vi "Load Sequence.vi"(8 "error in":errorcluster, 10 "path":path, 11 "Sequence Executor in":refnum<class "Sequence Executor.lvclass">) -> (0 "error out":errorcluster, 3 "Sequence Executor out":refnum<class "Sequence Executor.lvclass">)   [LabVIEW 2026, in "Sequence Executor.lvclass"]
doc: "Loads a sequence JSON and launches its rig plug-in. Refuses while Running. Reads and parses the sequence and rig config and validates them; any error or invalid sequence sets Status LOAD ERROR and returns NO error (AF would stop the actor). Otherwise stops the previous rig, loads the plug-in class, casts it to Rig, sets its config, launches it nested (auto-stop), and stores Sequence, Rig Config, Rig Enqueuer, Loaded, Results (all NOT RUN) and Status through the class accessors. A launch error also sets Status LOAD ERROR and Loaded F."
uses:
  Sequence Executor.lvclass
  Rig/Rig.lvclass
  Sequence Executor.lvclass/Sequence Executor.ctl
  <vilib>/ActorFramework/Message Enqueuer/Message Enqueuer.lvclass/Message Enqueuer.ctl
  <vilib>/ActorFramework/Message Enqueuer/Enqueue.vi
  <vilib>/ActorFramework/Stop Msg/Stop Msg.lvclass
  <vilib>/ActorFramework/Message Priority Queue/Priority Enqueue.vi
  <vilib>/ActorFramework/Message Enqueuer/Message Enqueuer.lvclass
  <vilib>/ActorFramework/Actor/Actor.lvclass
panel:
  in  "Rig type":refnum<class "Rig.lvclass">
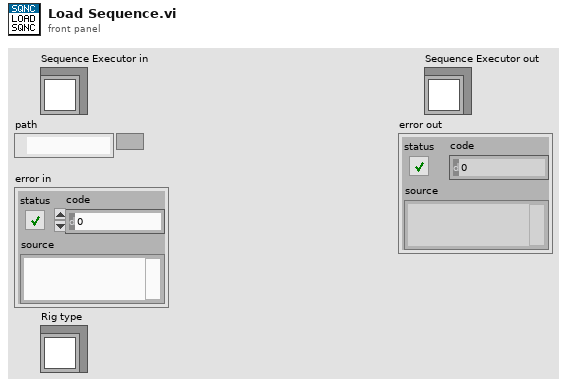
[diagram p1: front panel]
types:
  T1 = cluster{"step_no":i32, "step_name":string, "result":string, "reason":string, "measured":dbl, "target":dbl, "duration_ms":dbl}
  T2 = typedef "Sequence File.ctl" = cluster{"sequence_id":string, "description":string, "rig_config":string, "steps":T3[]}
  T3 = typedef "Step Config.ctl" = cluster{"step_no":i32, "step_name":string, "command_type":string, "setpoints":T4[], "conditions":T5[], "dwell_time_ms":i32, "timeout_ms":i32, "expected_result":string}
  T4 = typedef "Channel Value.ctl" = cluster{"channel":string, "value":dbl}
  T5 = typedef "Condition.ctl" = cluster{"channel":string, "target":dbl, "tolerance":dbl}
  T6 = typedef "Rig Config.ctl" = cluster{"rig_id":string, "description":string, "plugin_class":string, "channels":T7[]}
  T7 = typedef "Channel Definition.ctl" = cluster{"name":string, "unit":string, "min":dbl, "max":dbl}
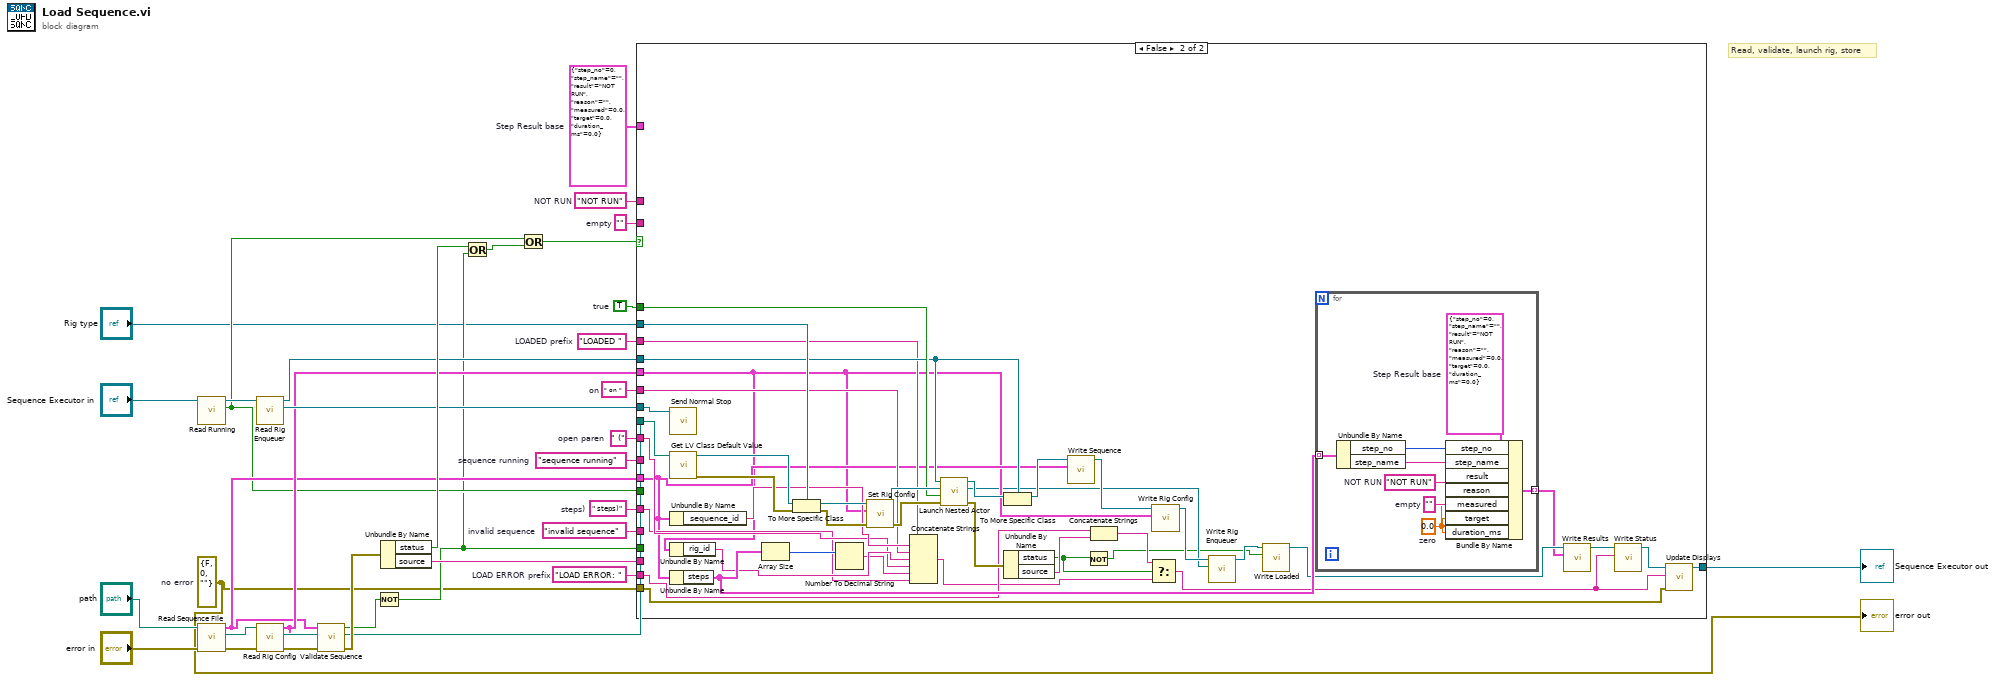
[diagram p0: block diagram]
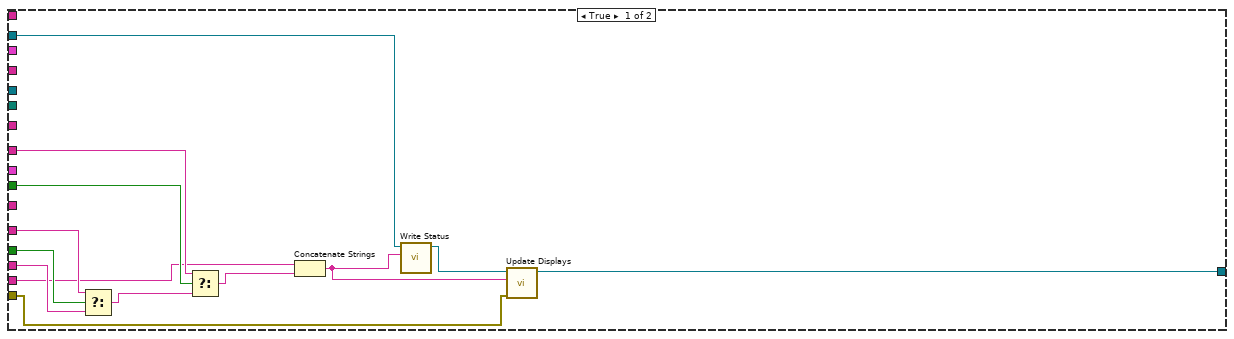
[diagram p2: hidden frame]
diagram:
  w11 = T1 {"step_no"=0, "step_name"="", "result"="NOT RUN", "reason"="", "measured"=0.0, "target"=0.0, "duration_ms"=0.0}  # Step Result base
  w12 = TRUE  # true
  w5 = " steps)"  # steps)
  w6 = " ("  # open paren
  w7 = " on "  # on
  w8 = "LOADED "  # LOADED prefix
  w9 = ""  # empty
  w10 = "NOT RUN"  # NOT RUN
  w15 = "invalid sequence"  # invalid sequence
  w14 = "sequence running"  # sequence running
  w13 = "LOAD ERROR: "  # LOAD ERROR prefix
  w3 = errorcluster {"status"=FALSE, "code"=0, "source"=""}  # no error
  # "Read, validate, launch rig, store"
  n1 = call "Read Running.vi"("Sequence Executor in"="Sequence Executor in") -> ("Running"=w17:bool, "Sequence Executor out"=w28:refnum<class "Sequence Executor.lvclass">)  [unwired: 8 in, 1 out]
  n2 = call "Read Sequence File.vi"("error in"="error in", "path"="path") -> ("error out"=w31:errorcluster, "rig config path"=w32:path, "Sequence File"=w19:T2)  [unwired: 7 in]
  n3 = call "Read Rig Enqueuer.vi"("Sequence Executor in"=w28) -> ("Actor Framework:Message Enqueuer"=w22:refnum<class "Message Enqueuer.lvclass">, "Sequence Executor out"=w23:refnum<class "Sequence Executor.lvclass">)  [unwired: 8 in, 1 out]
  n4 = call "Read Rig Config.vi"("error in"=w31, "path"=w32) -> ("error out"=w30:errorcluster, "plugin class path"=w21:path, "Rig Config"=w20:T6)  [unwired: 7 in]
  n5 = call "Validate Sequence.vi"("error in"=w30, "Rig Config"=w20, "Sequence File"=w19) -> ("error out"=w27:errorcluster, "valid"=w26:bool)  [unwired: 6 in, 1 out]
  n6 = Not(x=w26) -> (.not. x?=w16:bool)
  n7 = Unbundle By Name(w27) -> ("status"=w25:bool, "source"=w18:string)
  n8 = Or(x=w25, y=w16) -> (x .or. y?=w24:bool)
  n9 = Or(x=w17, y=w24) -> (x .or. y?=w1:bool)
  n10 = case shown="False" w1 {
    tunnel: w23 -> [w39 w78]
    tunnel: w22 -> [_ w89]
    tunnel: w21 -> [_ w88]
    tunnel: w20 -> [_ w59]
    tunnel: w19 -> [_ w61]
    tunnel: w18 -> [w45 _]
    tunnel: w17 -> [w44 _]
    tunnel: w16 -> [w47 _]
    tunnel: w15 -> [w46 _]
    tunnel: w14 -> [w43 _]
    tunnel: w13 -> [w41 w67]
    tunnel: w12 -> [_ w81]
    tunnel: w11 -> [_ _]
    tunnel: w10 -> [_ _]
    tunnel: w9 -> [_ _]
    tunnel: w8 -> [_ w75]
    tunnel: w7 -> [_ w73]
    tunnel: w6 -> [_ w71]
    tunnel: w5 -> [_ w69]
    tunnel: "Rig type" -> [_ w86]
    tunnel: w3 -> [w36 w49]
    tunnel: [w35 w48] -> w2
    frame True {
      n11 = Select(t=w46, s=w47, f=w45) -> (s? t:f=w42:string)
      n12 = Select(t=w43, s=w44, f=w42) -> (s? t:f=w40:string)
      n13 = Concatenate Strings(w41, w40) -> (w37:string)
      n14 = call "Write Status.vi"("Status"=w37, "Sequence Executor in"=w39) -> ("Sequence Executor out"=w38:refnum<class "Sequence Executor.lvclass">)  [unwired: 8 in, 1 out]
      n15 = call "Update Displays.vi"("error in"=w36, "Status"=w37, "Sequence Executor in"=w38) -> ("Sequence Executor out"=w35:refnum<class "Sequence Executor.lvclass">)  [unwired: 7 in, 1 out]
    }
    frame False {
      n16 = call <vilib>:"Send Normal Stop.vi"("Message Enqueuer"=w89) -> ()  [unwired: 10 in, 1 out]
      n17 = call <vilib>:"Get LV Class Default Value.vi"("class path"=w88) -> ("error out"=w85:errorcluster, "object"=w87:refnum<class>)  [unwired: 9 in]
      n18 = Unbundle By Name(w61) -> ("sequence_id"=w74:string)
      n19 = Unbundle By Name(w59) -> ("rig_id"=w72:string)
      n20 = Unbundle By Name(w61) -> ("steps"=w77:T3[])
      n21 = Array Size(array=w77) -> (size(s)=w76:i32)
      n22 = To More Specific Class(target class=w86, reference=w87, error in=w85) -> (specific class reference=w84:refnum<class "Rig.lvclass">, error out=w83:errorcluster)
      n23 = Number To Decimal String(number=w76) -> (decimal integer string=w70:string)  [unwired: 1 in]
      n24 = call "Set Rig Config.vi"("error in"=w83, "Rig Config"=w59, "Rig in"=w84) -> ("error out"=w80:errorcluster, "Rig out"=w82:refnum<class "Rig.lvclass">)  [unwired: 7 in]
      n25 = Concatenate Strings(w75, w74, w73, w72, w71, w70, w69) -> (w64:string)
      n26 = call <vilib>:"Launch Nested Actor.vi"("error in (no error)"=w80, "Auto-stop? (T)"=w81, "Nested Actor"=w82, "Caller Actor in"=w78) -> ("error out"=w68:errorcluster, "Nested Actor's Enqueuer"=w57:refnum<class "Message Enqueuer.lvclass">, "Caller Actor out"=w79:refnum<class "Sequence Executor.lvclass">)  [unwired: 5 in]
      n27 = To More Specific Class(target class=w78, reference=w79) -> (specific class reference=w62:refnum<class "Sequence Executor.lvclass">)  [unwired: 1 in, 1 out]
      n28 = Unbundle By Name(w68) -> ("status"=w63:bool, "source"=w66:string)
      n29 = call "Write Sequence.vi"("Sequence File"=w61, "Sequence Executor in"=w62) -> ("Sequence Executor out"=w60:refnum<class "Sequence Executor.lvclass">)  [unwired: 8 in, 1 out]
      n30 = Not(x=w63) -> (.not. x?=w55:bool)
      n31 = Concatenate Strings(w67, w66) -> (w65:string)
      n32 = Select(t=w65, s=w63, f=w64) -> (s? t:f=w50:string)
      n33 = call "Write Rig Config.vi"("Rig Config"=w59, "Sequence Executor in"=w60) -> ("Sequence Executor out"=w58:refnum<class "Sequence Executor.lvclass">)  [unwired: 8 in, 1 out]
      n34 = call "Write Rig Enqueuer.vi"("Actor Framework:Message Enqueuer"=w57, "Sequence Executor in"=w58) -> ("Sequence Executor out"=w56:refnum<class "Sequence Executor.lvclass">)  [unwired: 8 in, 1 out]
      n35 = call "Write Loaded.vi"("Loaded"=w55, "Sequence Executor in"=w56) -> ("Sequence Executor out"=w54:refnum<class "Sequence Executor.lvclass">)  [unwired: 8 in, 1 out]
      n36 = for {
        tunnel: w77 -> [w97] mode=indexing
        tunnel: [w90] -> w53 mode=indexing
        w93 = ""  # empty
        w94 = "NOT RUN"  # NOT RUN
        w91 = T1 {"step_no"=0, "step_name"="", "result"="NOT RUN", "reason"="", "measured"=0.0, "target"=0.0, "duration_ms"=0.0}  # Step Result base
        w92 = 0.0  # zero
        n37 = Unbundle By Name(w97) -> ("step_no"=w96:i32, "step_name"=w95:string)
        n38 = Bundle By Name(cluster=w91, "step_no"=w96, "step_name"=w95, "result"=w94, "reason"=w93, "measured"=w92, "target"=w92, "duration_ms"=w92) -> (w90:T1)
      }
      n39 = call "Write Results.vi"("Results"=w53, "Sequence Executor in"=w54) -> ("Sequence Executor out"=w52:refnum<class "Sequence Executor.lvclass">)  [unwired: 8 in, 1 out]
      n40 = call "Write Status.vi"("Status"=w50, "Sequence Executor in"=w52) -> ("Sequence Executor out"=w51:refnum<class "Sequence Executor.lvclass">)  [unwired: 8 in, 1 out]
      n41 = call "Update Displays.vi"("error in"=w49, "Status"=w50, "Sequence Executor in"=w51) -> ("Sequence Executor out"=w48:refnum<class "Sequence Executor.lvclass">)  [unwired: 7 in, 1 out]
    }
  }
  "Sequence Executor out" <- w2
  "error out" <- w3
